vi "Update Configuration Control.vi"(8 "error in (no error)":errorcluster, 9 "Configuration in":T1={"Common"={"Period (s)"=0.001, "Offset (us)"=0, "Priority"=100, "Processor"=-2, "External Clock"={"ClockID"=0, "Clock Name"="", "Publish Clock"=FALSE, "Convert Data Timestamps"=FALSE, "Plugin Timing Source"=FALSE}}, "TX Interface"="CAN2", "Port Configuration"={"Mode"=enum."CAN FD", "Baud Rate"=500000, "Temination On"=TRUE, "Subordinate"=FALSE, "Echo TX"=FALSE, "FD Config"={"FD Baud Rate"=2000000, "ISO Mode"=TRUE, "BRS Enabled"=TRUE}}, "Filter"={"Allow List (ID)"=[], "Deny List (ID)"=[]}, "Wake Offset (us)"=100, "One Shot"=FALSE} {"Filter"."Deny List (ID)" format="%.0x"; "Filter"."Allow List (ID)" format="%.0x"; "Port Configuration"."FD Config"."FD Baud Rate" format="%.0p"; "Port Configuration"."Baud Rate" format="%.0p"; "Common"."Period (s)" format="%#_13g"}, 10 "Not Valid":bool, 11 "JSON Configuration":string) -> (0 "error out":errorcluster, 1 "Configuration out":T1={"Common"={"Period (s)"=0.001, "Offset (us)"=0, "Priority"=100, "Processor"=-2, "External Clock"={"ClockID"=0, "Clock Name"="", "Publish Clock"=FALSE, "Convert Data Timestamps"=FALSE, "Plugin Timing Source"=FALSE}}, "TX Interface"="CAN2", "Port Configuration"={"Mode"=enum."CAN FD", "Baud Rate"=500000, "Temination On"=TRUE, "Subordinate"=FALSE, "Echo TX"=FALSE, "FD Config"={"FD Baud Rate"=2000000, "ISO Mode"=TRUE, "BRS Enabled"=TRUE}}, "Filter"={"Allow List (ID)"=[], "Deny List (ID)"=[]}, "Wake Offset (us)"=100, "One Shot"=FALSE} {"Filter"."Deny List (ID)" format="%.0x"; "Filter"."Allow List (ID)" format="%.0x"; "Port Configuration"."FD Config"."FD Baud Rate" format="%.0p"; "Port Configuration"."Baud Rate" format="%.0p"; "Common"."Period (s)" format="%#_13g"})   [LabVIEW 2021, in "CIF CAN_Writer_NIXNET UI.lvlib"]
uses:
  CIF CAN_Writer_NIXNET UI.lvlib
  Common/Typedef/Configuration.ctl
  <vilib>/CIF Foundation/CIF Core/CIFCore/Common/Typedef/Common Plugin Configuration.ctl
  <vilib>/CIF Foundation/CIF Core/CIFCore/Common/Typedef/External Clock Config.ctl
  <vilib>/CIF Foundation/CIF CAN RW Core/typedef/CAN Port Configuration.ctl
  <vilib>/CIF Foundation/CIF CAN RW Core/typedef/CAN Mode.ctl
  <vilib>/CIF Foundation/CIF CAN RW Core/typedef/FD Config.ctl
  <vilib>/CIF Foundation/CIF CAN RW Core/typedef/CAN Filter.ctl
  <vilib>/addons/_JKI.lib/Serialization/JSON/JKI JSON Serialization.lvlib
  <vilib>/CIF Foundation/CIF Core/CIFCore/Common/CIFCoreCommon.lvlib
  Common/CAN_Writer_NIXNET_Common.lvlib
  <vilib>/CIF Foundation/CIF CAN RW Core/CAN_RW_CORE.lvclass
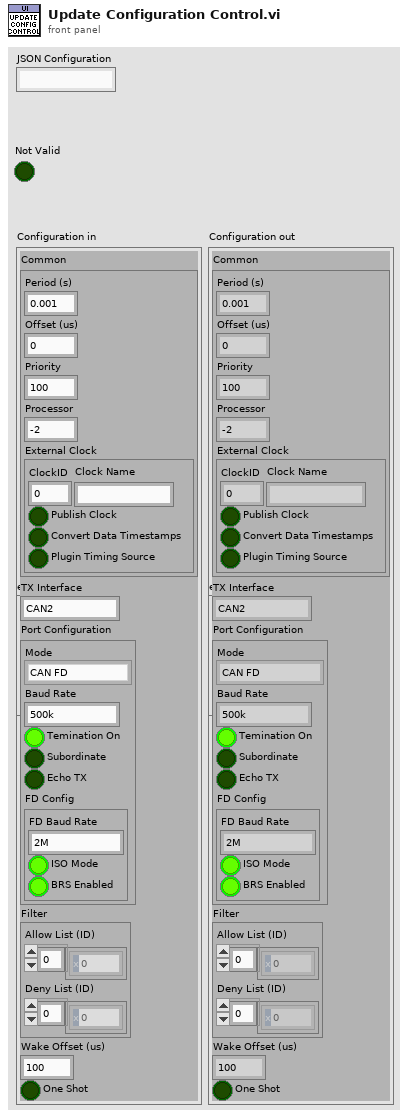
[diagram p1: front panel]
types:
  T1 = typedef "CAN_Writer_NIXNET_Common.lvlib/Configuration.ctl" = cluster{"Common":T2, "TX Interface":string, "Port Configuration":T4, "Filter":T7, "Wake Offset (us)":i64, "One Shot":bool}
  T2 = typedef "CIFCoreCommon.lvlib/Common Plugin Configuration.ctl" = cluster{"Period (s)":dbl, "Offset (us)":i32, "Priority":i32, "Processor":i32, "External Clock":T3}
  T3 = typedef "CIFCoreCommon.lvlib/External Clock Config.ctl" = cluster{"ClockID":u8, "Clock Name":string, "Publish Clock":bool, "Convert Data Timestamps":bool, "Plugin Timing Source":bool}
  T4 = typedef "CAN_RW_CORE.lvclass/CAN Port Configuration.ctl" = cluster{"Mode":T5, "Baud Rate":u64, "Temination On":bool, "Subordinate":bool, "Echo TX":bool, "FD Config":T6}
  T5 = typedef "CAN_RW_CORE.lvclass/CAN Mode.ctl" = enum16{"CAN 2.0", "CAN FD"}
  T6 = typedef "CAN_RW_CORE.lvclass/FD Config.ctl" = cluster{"FD Baud Rate":u64, "ISO Mode":bool, "BRS Enabled":bool}
  T7 = typedef "CAN_RW_CORE.lvclass/CAN Filter.ctl" = cluster{"Allow List (ID)":u32[], "Deny List (ID)":u32[]}
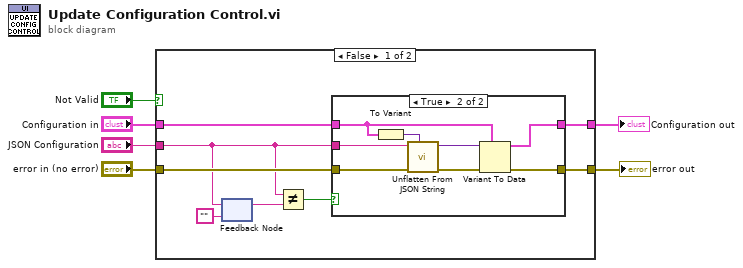
[diagram p0: block diagram]
diagram:
  n1 = case shown="False" "Not Valid" {
    tunnel: [w14 w26] -> w3
    tunnel: "error in (no error)" -> [w13 w26]
    tunnel: "Configuration in" -> [w8 w25]
    tunnel: "JSON Configuration" -> [w11 _]
    tunnel: [w7 w25] -> w1
    frame False {
      n2 = feedback #1("" ("JSON Configuration")) -> (w10:string)
      n3 = feedback-in #1(w11) -> ()
      n4 = Not Equal?(x=w11, y=w10) -> (x != y?=w9:bool)
      n5 = case shown="True" w9 {
        tunnel: [w16 w18] -> w14
        tunnel: w13 -> [w16 w20]
        tunnel: w11 -> [_ w23]
        tunnel: w8 -> [w15 w19]
        tunnel: [w15 w17] -> w7
        frame False {
        }
        frame True {
          n6 = To Variant(anything=w19) -> (Variant=w21:variant)
          n7 = call <vilib>:"Unflatten From JSON String.vi"("Type and Defaults"=w21, "error in"=w20, "JSON String"=w23) -> ("error out"=w22:errorcluster, "Variant"=w24:variant)  [unwired: 7 in]
          n8 = Variant To Data(error in=w22, type=w19, Variant=w24) -> (data=w17:T1, error out=w18:errorcluster)
        }
      }
    }
    frame True {
    }
  }
  "error out" <- w3
  "Configuration out" <- w1
